vi "Reflection Native Read Property Value.vi"(8 "error in (no error)":errorcluster, 10 "Target Object":refnum<k24>, 11 "Property Info in":refnum<k24>) -> (0 "error out":errorcluster, 2 "Property Value":refnum<k24>, 3 "Property Info out":refnum<k24>)   [LabVIEW 2026, in "ToastNotification.lvlib" / "Reflection DotNet.lvlib"]
doc: "Native PropertyInfo.GetValue overload with no index arguments. Borrow Property Info in and Target Object. Property Value is an acquired boxed result; caller closes it after use even on an error path. Property Info out aliases the metadata input. Indexed properties require another overload."
uses:
  Reflection DotNet.lvlib
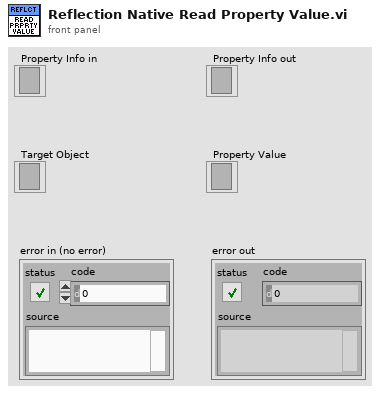
[diagram p1: front panel]
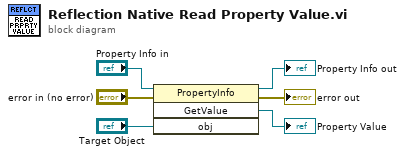
[diagram p0: block diagram]
diagram:
  n1 = invoke class="PropertyInfo" method="GetValue"(reference="Property Info in", error in="error in (no error)", "obj"="Target Object") -> (reference out=→"Property Info out":refnum<k24>, error out=→"error out":errorcluster, "GetValue"=→"Property Value":refnum<k24>)  [unwired: 1 in, 1 out]
